vi "WriteSensorMake.vi"(8 "Error In":errorcluster, 10 "SensorMake":T1, 11 "object in":refnum<class "Controller.lvclass">) -> (0 "Error Out":errorcluster, 3 "object out":refnum<class "Controller.lvclass">)   [LabVIEW 2022 SP3, in "Controller.lvlib" / "Controller.lvclass"]
uses:
  Controller.lvclass
  TypeDef/SensorMake.ctl
  Controller.lvclass/Controller.ctl
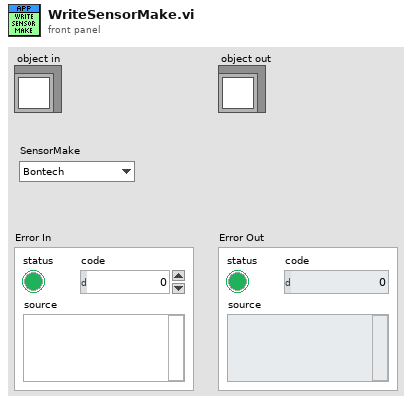
[diagram p1: front panel]
types:
  T1 = typedef "SensorMake.ctl" = enum16{"Bontech", "DTImaging", "VarexImaging"}
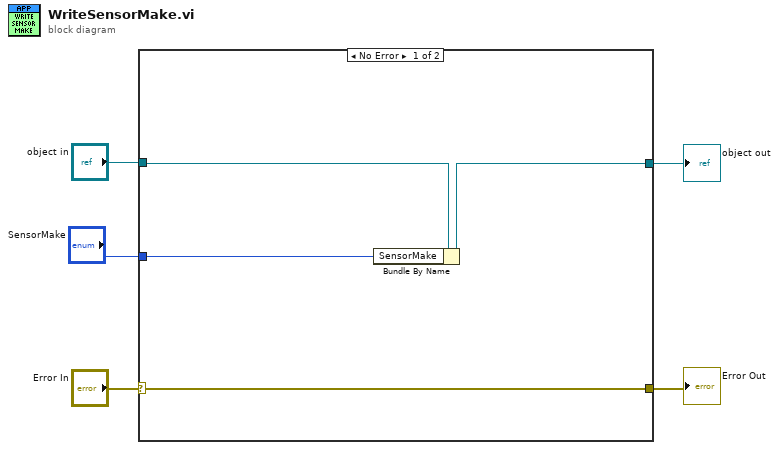
[diagram p0: block diagram]
diagram:
  n1 = case shown="No Error" "Error In" {
    selector: "Error In" -> [w8 w11]
    tunnel: [w8 w11] -> w4
    tunnel: [w6 w10] -> w2
    tunnel: "object in" -> [w7 w10]
    tunnel: "SensorMake" -> [w9 _]
    frame No Error {
      n2 = Bundle By Name(cluster=w7, "SensorMake"=w9) -> (w6:refnum<class "Controller.lvclass">)
    }
    frame Error {
    }
  }
  "Error Out" <- w4
  "object out" <- w2
